vi "LabVIEW.Elements.Write API Name and Status.vi"(7 "Command":T1, 8 "Fehler (Eingang, kein Fehler)":errorcluster, 10 "Status[]":bool[](array[boolean]), 11 "Array Reference":refnum<vi>) -> (0 "Fehler (Ausgang)":errorcluster)   [LabVIEW 2019]
uses:
  LabVIEW.Type Definitions/LabVIEW.Main.Main_Program_Command.ctl
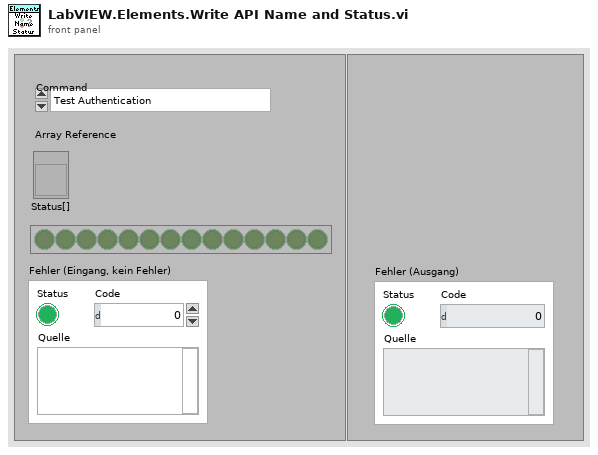
[diagram p1: front panel]
types:
  T1 = typedef "LabVIEW.Main.Main_Program_Command.ctl" = enum16{"Test Authentication", "Test Label", "Test Product/Serial Number", "Test Vorgang/Fertigmeldung", "Test User"}
  T2 = cluster{"API Name":string, "API":string, "LED":bool}
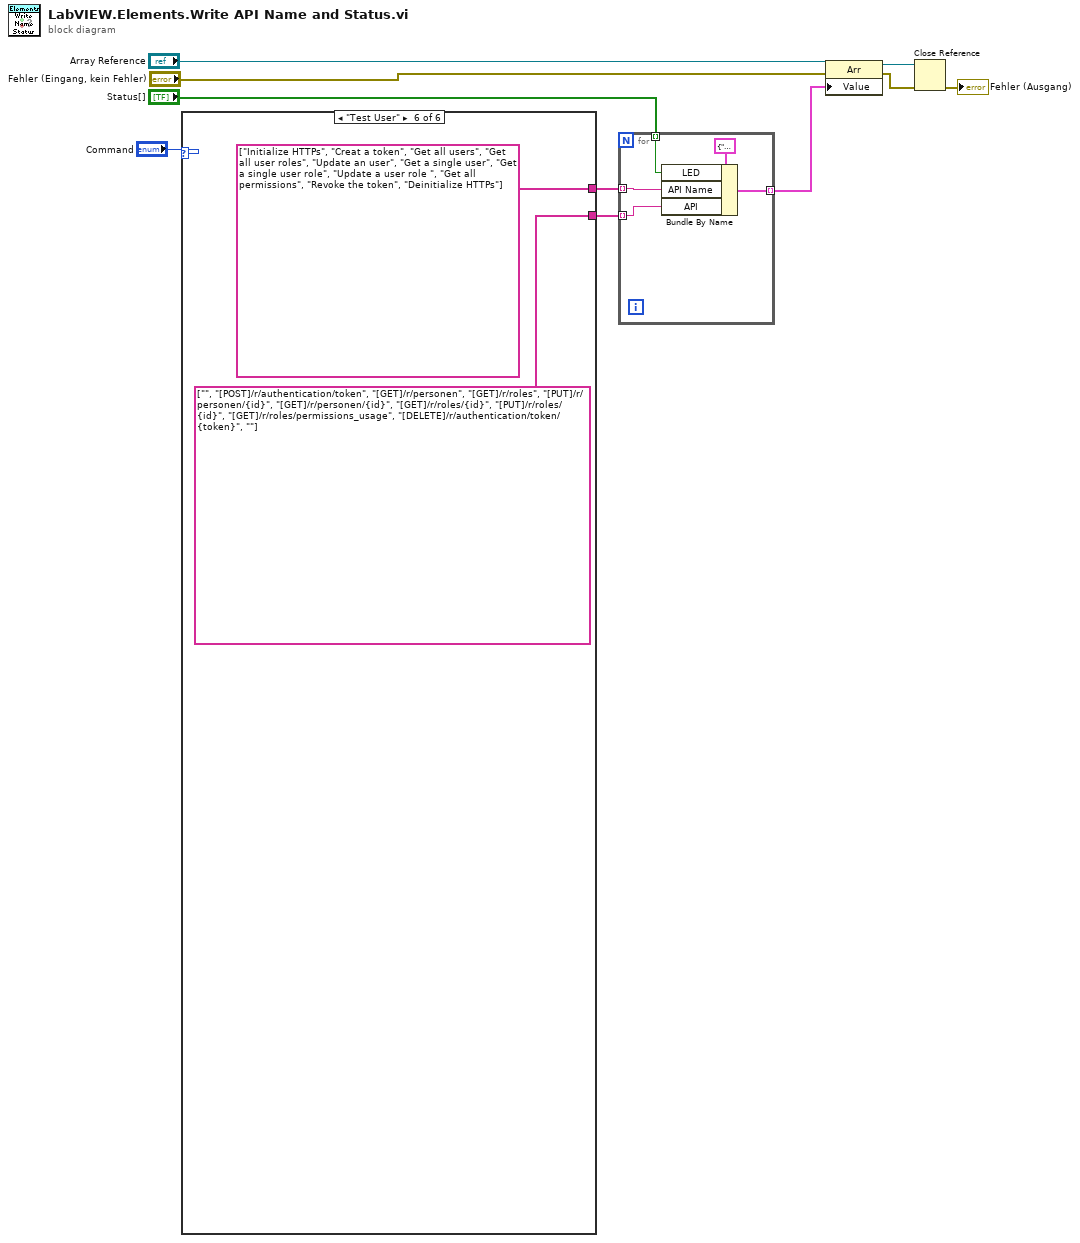
[diagram p0: block diagram]
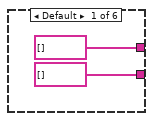
[diagram p2: hidden frame]
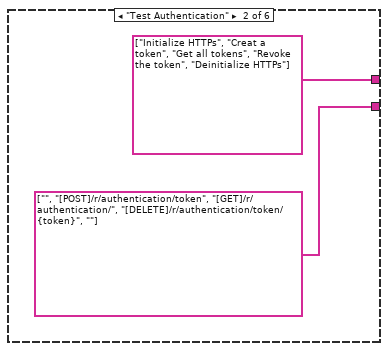
[diagram p3: hidden frame]
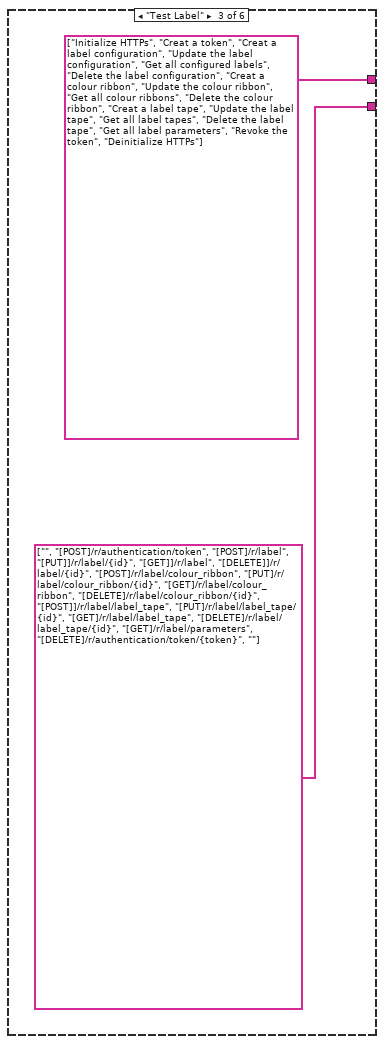
[diagram p4: hidden frame]
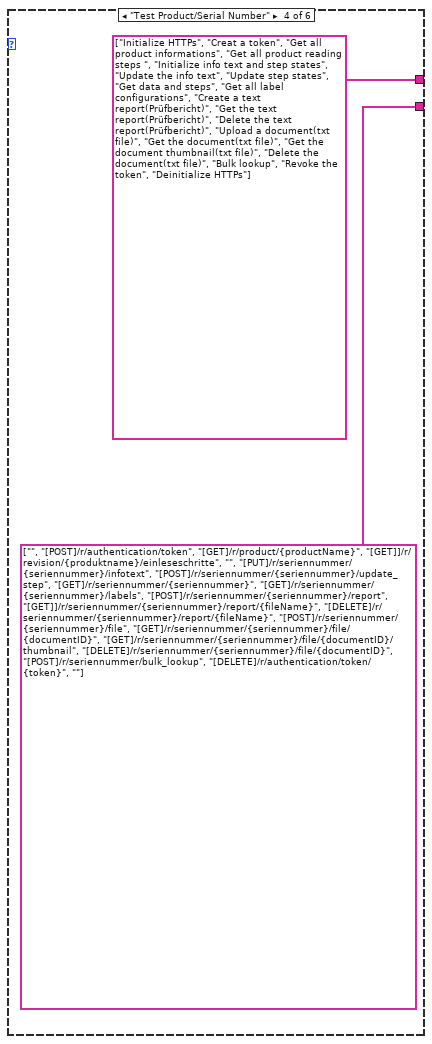
[diagram p5: hidden frame]
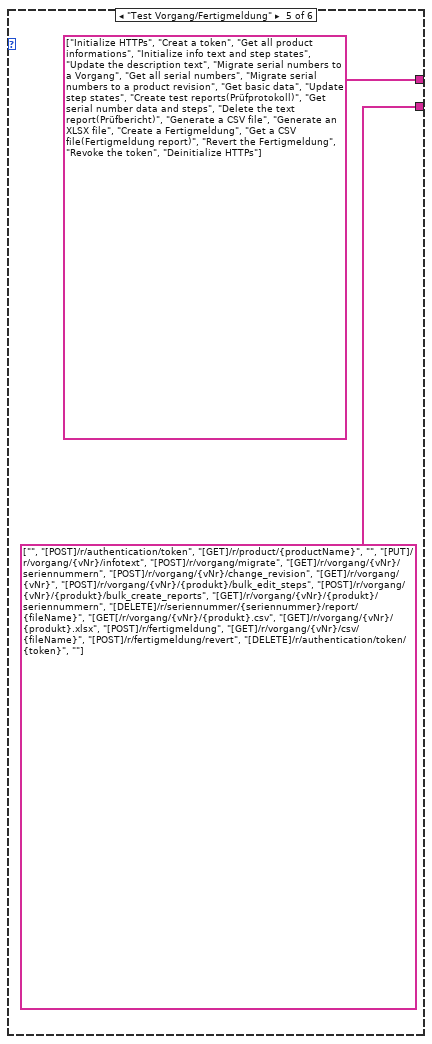
[diagram p6: hidden frame]
diagram:
  n1 = case shown="\"Test User\"" "Command" {
    tunnel: [string[] [] string[] ["Initialize HTTPs", "Creat a token", "Get all tokens", "Revoke the token", "Deinitialize HTTPs"] string[] ["Initialize HTTPs", "Creat a token", "Creat a label configuration", "Update the label configuration", "Get all configured labels", "Delete the label configuration", "Creat a colour ribbon", "Update the colour ribbon", "Get all colour ribbons", "Delete the colour ribbon", "Creat a label tape", "Update the label tape", "Get all label tapes", "Delete the label tape", "Get all label parameters", "Revoke the token", "Deinitialize HTTPs"] string[] ["Initialize HTTPs", "Creat a token", "Get all product informations", "Get all product reading steps ", "Initialize info text and step states", "Update the info text", "Update step states", "Get data and steps", "Get all label configurations", "Create a text report(Prüfbericht)", "Get the text report(Prüfbericht)", "Delete the text report(Prüfbericht)", "Upload a document(txt file)", "Get the document(txt file)", "Get the document thumbnail(txt file)", "Delete the document(txt file)", "Bulk lookup", "Revoke the token", "Deinitialize HTTPs"] string[] ["Initialize HTTPs", "Creat a token", "Get all product informations", "Initialize info text and step states", "Update the description text", "Migrate serial numbers to a Vorgang", "Get all serial numbers", "Migrate serial numbers to a product revision", "Get basic data", "Update step states", "Create test reports(Prüfprotokoll)", "Get serial number data and steps", "Delete the text report(Prüfbericht)", "Generate a CSV file", "Generate an XLSX file", "Create a Fertigmeldung", "Get a CSV file(Fertigmeldung report)", "Revert the Fertigmeldung", "Revoke the token", "Deinitialize HTTPs"] string[] ["Initialize HTTPs", "Creat a token", "Get all users", "Get all user roles", "Update an user", "Get a single user", "Get a single user role", "Update a user role ", "Get all permissions", "Revoke the token", "Deinitialize HTTPs"]] -> w9
    tunnel: [string[] [] string[] ["", "[POST]/r/authentication/token", "[GET]/r/authentication/", "[DELETE]/r/authentication/token/{token}", ""] string[] ["", "[POST]/r/authentication/token", "[POST]/r/label", "[PUT]]/r/label/{id}", "[GET]]/r/label", "[DELETE]]/r/label/{id}", "[POST]/r/label/colour_ribbon", "[PUT]/r/label/colour_ribbon/{id}", "[GET]/r/label/colour_ribbon", "[DELETE]/r/label/colour_ribbon/{id}", "[POST]]/r/label/label_tape", "[PUT]/r/label/label_tape/{id}", "[GET]/r/label/label_tape", "[DELETE]/r/label/label_tape/{id}", "[GET]/r/label/parameters", "[DELETE]/r/authentication/token/{token}", ""] string[] ["", "[POST]/r/authentication/token", "[GET]/r/product/{productName}", "[GET]]/r/revision/{produktname}/einleseschritte", "", "[PUT]/r/seriennummer/{seriennummer}/infotext", "[POST]/r/seriennummer/{seriennummer}/update_step", "[GET]/r/seriennummer/{seriennummer}", "[GET]/r/seriennummer/{seriennummer}/labels", "[POST]/r/seriennummer/{seriennummer}/report", "[GET]]/r/seriennummer/{seriennummer}/report/{fileName}", "[DELETE]/r/seriennummer/{seriennummer}/report/{fileName}", "[POST]/r/seriennummer/{seriennummer}/file", "[GET]/r/seriennummer/{seriennummer}/file/{documentID}", "[GET]/r/seriennummer/{seriennummer}/file/{documentID}/thumbnail", "[DELETE]/r/seriennummer/{seriennummer}/file/{documentID}", "[POST]/r/seriennummer/bulk_lookup", "[DELETE]/r/authentication/token/{token}", ""] string[] ["", "[POST]/r/authentication/token", "[GET]/r/product/{productName}", "", "[PUT]/r/vorgang/{vNr}/infotext", "[POST]/r/vorgang/migrate", "[GET]/r/vorgang/{vNr}/seriennummern", "[POST]/r/vorgang/{vNr}/change_revision", "[GET]/r/vorgang/{vNr}", "[POST]/r/vorgang/{vNr}/{produkt}/bulk_edit_steps", "[POST]/r/vorgang/{vNr}/{produkt}/bulk_create_reports", "[GET]/r/vorgang/{vNr}/{produkt}/seriennummern", "[DELETE]/r/seriennummer/{seriennummer}/report/{fileName}", "[GET[/r/vorgang/{vNr}/{produkt}.csv", "[GET]/r/vorgang/{vNr}/{produkt}.xlsx", "[POST]/r/fertigmeldung", "[GET]/r/vorgang/{vNr}/csv/{fileName}", "[POST]/r/fertigmeldung/revert", "[DELETE]/r/authentication/token/{token}", ""] string[] ["", "[POST]/r/authentication/token", "[GET]/r/personen", "[GET]/r/roles", "[PUT]/r/personen/{id}", "[GET]/r/personen/{id}", "[GET]/r/roles/{id}", "[PUT]/r/roles/{id}", "[GET]/r/roles/permissions_usage", "[DELETE]/r/authentication/token/{token}", ""]] -> w8
    frame Default {
    }
    frame "Test Authentication" {
    }
    frame "Test Label" {
    }
    frame "Test Product/Serial Number" {
    }
    frame "Test Vorgang/Fertigmeldung" {
    }
    frame "Test User" {
    }
  }
  n2 = for {
    tunnel: w9 -> [w26] mode=indexing
    tunnel: w8 -> [w25] mode=indexing
    tunnel: "Status[]" -> [w24] mode=indexing
    tunnel: [w23] -> w6 mode=indexing
    n3 = Bundle By Name(cluster=T2 {"API Name"="", "API"="", "LED"=FALSE} ("API Status Cluster"), "LED"=w24, "API Name"=w26, "API"=w25) -> (w23:T2)
  }
  n4 = property class="Arr"(reference="Array Reference", error in="Fehler (Eingang, kein Fehler)", "Value"=w6) -> (reference out=w5:refnum<vi>, error out=w4:errorcluster)
  n5 = Close Reference(reference=w5, error in (no error)=w4) -> (error out=→"Fehler (Ausgang)":errorcluster)
